vi "登录.vi"() -> ()   [LabVIEW 2026]
doc: "系统登录界面 - APS 测控软件 临时台设备侧。仅前面板布局演示，无程序逻辑。来源：登录.html 主界面。"
panel:
  out "13 状态栏-授权":string="授权: --"
  out "12 状态栏-登录状态":string="登录状态: 未登录"
  out "11 状态栏-版本":string="版本: V2.4.1"
  out "10 状态栏-系统":string="系统: APS 设备侧计量"
  out "09 网络状态":string="● 链路就绪"
  in  "申请账号":bool
  in  "忘记密码":bool
  in  "取消按钮":bool
  in  "登录按钮":bool
  in  "记住密码":bool
  in  "权限级别":i32(ring) items=["请选择登录角色", "系统管理员（Admin）", "测试工程师（Engineer）", "普通操作员（Operator）", "访客模式（Guest）"]
  in  "密码":string
  in  "用户名":string
  out "08 表单副题":string="欢迎回来，请输入您的账号信息"
  out "07 表单标题":string="系统登录"
  out "06 面板头":string="身份验证 | 请输入账号信息"
  out "05 版本徽标":string="Version 2.4.1"
  out "04 品牌英文":string="APS Temporary Station - Equipment Side Test and Control System"
  out "03 品牌标题":string="APS 测控软件"
  out "02 时钟":string="--:--:--"
  out "01 标题栏":string="● 系统登录 | APS 测控软件 · 临时台设备侧"
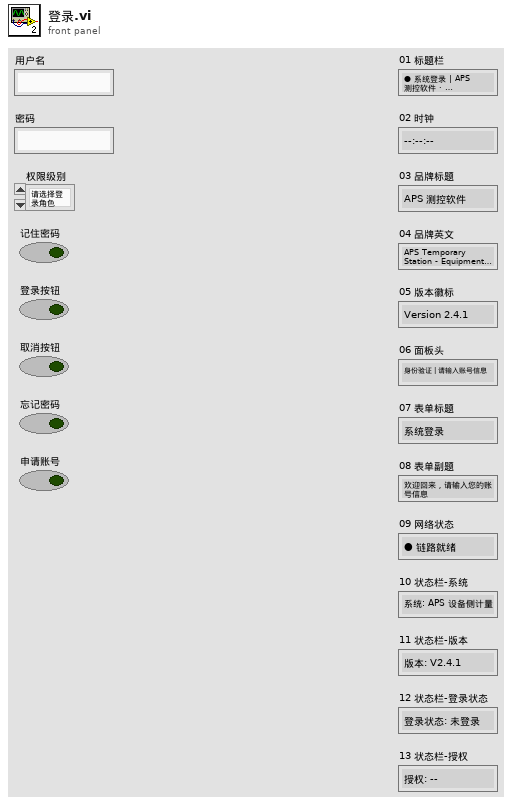
[diagram p1: front panel]
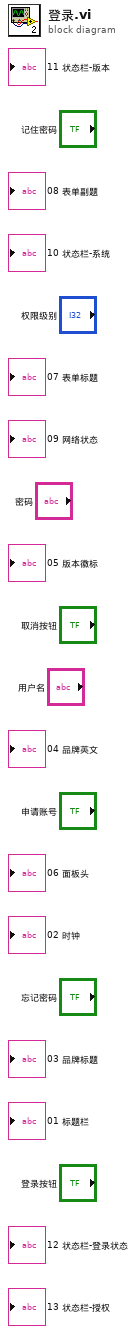
[diagram p0: block diagram]
diagram:
